vi "VIH - VI Doc Editor #2 - GenObject Symbols.vi"(6 "cmd (nop)":T2(ring), 8 "error in":errorcluster, 9 "type":enum16{"<Invalid>", "Control", "Page"}(ring), 11 "Gen Refnum":refnum<vi>) -> (0 "error out":errorcluster, 1 "Symbols":T1[](array[typedef]), 2 "Symbol Index":i32, 3 "dup Gen Refnum":refnum<vi>)   [LabVIEW 2014]
doc: "::: VI Helpeks :::\nCopyright (c) 2000-2026 Konstantin Shifershteyn. All rights reserved."
uses:
  <vilib>/picture/picture.llb/imagedata.ctl
panel:
  out "max Symbol Index":i32
  # "VI Helpeks\nCopyright (c) 2012-2026 Konstantin Shifershteyn"
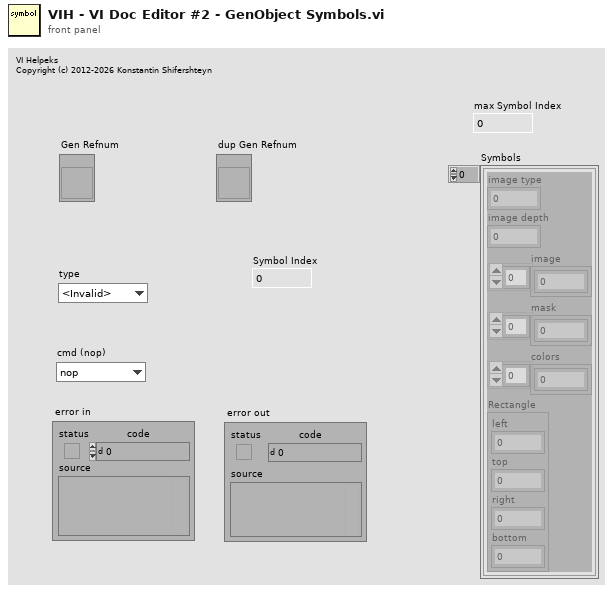
[diagram p1: front panel]
types:
  T1 = typedef "imagedata.ctl" = cluster{"image type":i32, "image depth":i32, "image":u8[], "mask":u8[], "colors":u32[], "Rectangle":cluster{"left":i16, "top":i16, "right":i16, "bottom":i16}}
  T2 = enum16{"nop", "Init", "get index", "get symbols"}
  T3 = cluster{"DefVal":variant, "Indicator":bool, i32}[]
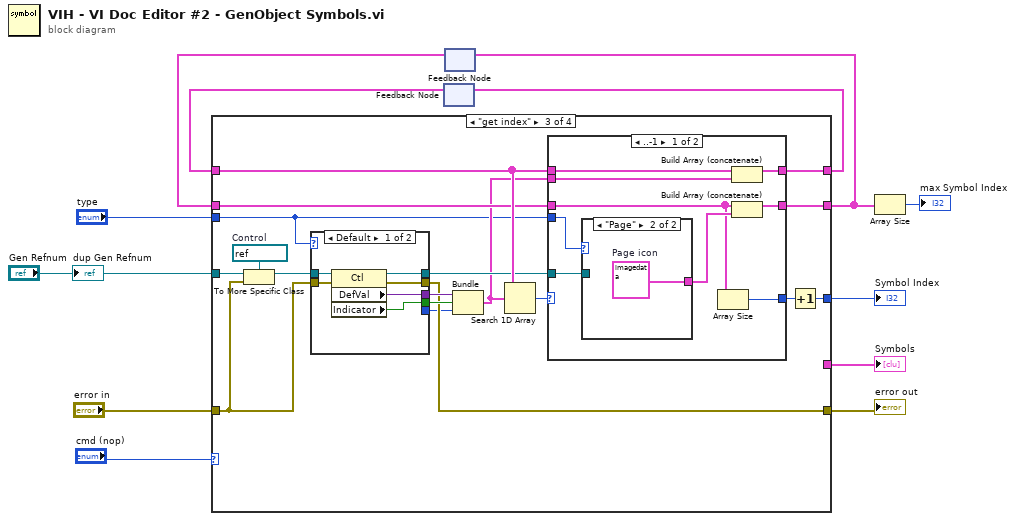
[diagram p0: block diagram]
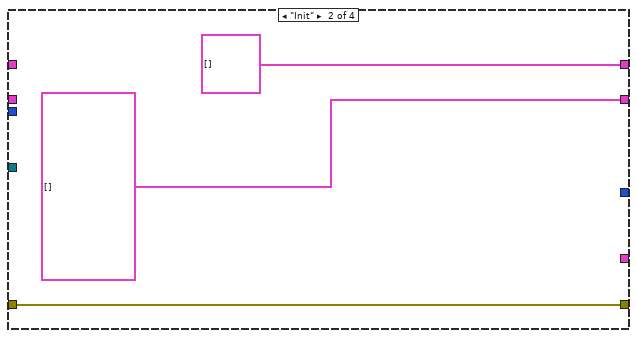
[diagram p3: hidden frame]
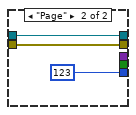
[diagram p4: hidden frame]
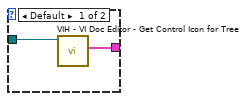
[diagram p5: hidden frame]
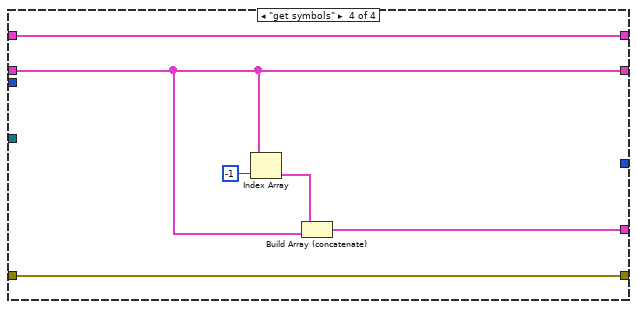
[diagram p7: hidden frame]
diagram:
  n1 = feedback #1() -> (w11:T3)  [unwired: 1 in]
  n2 = feedback #2() -> (w10:T1[])  [unwired: 1 in]
  n3 = case shown="\"get index\"" "cmd (nop)" {
    tunnel: [w15 T3 [] w36 w66] -> w12
    tunnel: w11 -> [w15 _ w35 w66]
    tunnel: w10 -> [w14 _ w34 w64]
    tunnel: [w14 T1[] [] w33 w64] -> w9
    tunnel: "Gen Refnum" -> [_ _ w22 _]
    tunnel: [_ _ w25 _] -> w7
    tunnel: [_ _ _ w62] -> w5
    tunnel: "error in" -> [w13 w17 w20 w61]
    tunnel: [w13 w17 w26 w61] -> w3
    tunnel: "type" -> [_ _ w19 _]
    frame "nop" {
    }
    frame "Init" {
    }
    frame "get index" {
      w23 = refnum<vi> refnum  # Control
      n4 = To More Specific Class(target class=w23, reference=w22, error in=w20) -> (specific class reference=w21:refnum<vi>)  [unwired: 1 out]
      n5 = case shown="Default" w19 {
        tunnel: [w42 w45] -> w31
        tunnel: [w41 _] -> w29
        tunnel: [w40 _] -> w28
        tunnel: [w39 w44] -> w26
        tunnel: w21 -> [w38 w45]
        tunnel: w20 -> [w37 w44]
        tunnel: [_ 123] -> w24
        frame Default {
          n6 = property class="Ctl"(reference=w38, error in=w37) -> (reference out=w42:refnum<vi>, error out=w39:errorcluster, "DefVal"=w41:variant, "Indicator"=w40:bool)
        }
        frame "Page" {
        }
      }
      n7 = Bundle("DefVal"=w29, "Indicator"=w28, w24) -> (w30:cluster{"DefVal":variant, "Indicator":bool, i32})  [unwired: 1 in]
      n8 = Search 1D Array(1D array=w35, element=w30) -> (index of element=w32:i32)  [unwired: 1 in]
      n9 = case shown="..-1" w32 {
        selector: w32 -> [_ w59]
        tunnel: [w53 w60] -> w36
        tunnel: w35 -> [w54 w60]
        tunnel: w30 -> [w52 _]
        tunnel: [w49 w59] -> w27
        tunnel: [w48 w58] -> w33
        tunnel: w34 -> [w47 w58]
        tunnel: w31 -> [w51 _]
        tunnel: w19 -> [w46 _]
        frame ..-1 {
          n10 = case shown="\"Page\"" w46 {
            tunnel: w51 -> [w56 _]
            tunnel: [w55 w57] -> w50
            frame Default {
              n11 = call "VIH - VI Doc Editor - Get Control Icon for Tree.vi"("Ctl Refnum"=w56) -> ("Icon"=w55:T1)  [unwired: 6 in, 4 out]
            }
            frame "Page" {
              w57 = T1 {"image type"=0, "image depth"=24, "image"=array[3072 elements], "mask"=[63, 254, 0, 0, 63, 255, 0, 0, 127, 255, 128, 0, 127, 255, 128, 0, 255, 255, 255, 252, 255, 255, 255, 254, 255, 255, 255, 255, 255, 255, 255, 255, 255, 255, 255, 255, 255, 255, 255, 255, 255, 255, 255, 255, 255, 255, 255, 255, 255, 255, 255, 255, 255, 255, 255, 255, 255, 255, 255, 255, 255, 255, 255, 255, 255, 255, 255, 255, 255, 255, 255, 255, 255, 255, 255, 255, 255, 255, 255, 255, 255, 255, 255, 255, 255, 255, 255, 255, 255, 255, 255, 255, 127, 255, 255, 254, 0, 0, 0, 0, 0, 0, 0, 0, 0, 0, 0, 0, 0, 0, 0, 0, 0, 0, 0, 0, 0, 0, 0, 0, 0, 0, 0, 0, 0, 0, 0, 0], "colors"=[], "Rectangle"={"left"=0, "top"=0, "right"=32, "bottom"=32}}  # Page icon
            }
          }
          n12 = Array Size(array=w47) -> (size(s)=w49:i32)
          n13 = Build Array (concatenate)(w54, w52) -> (w53:T3)
          n14 = Build Array (concatenate)(w47, w50) -> (w48:T1[])
        }
        frame 0.. {
        }
      }
      n15 = Increment(x=w27) -> (x+1=w25:i32)
    }
    frame "get symbols" {
      n16 = Index Array(array=w64, index=-1) -> (element=w63:T1)
      n17 = Build Array (concatenate)(w63, w64) -> (w62:T1[])
    }
  }
  "error out" <- w3
  "Symbol Index" <- w7
  "Symbols" <- w5
  n18 = feedback-in #1(w12) -> ()
  n19 = feedback-in #2(w9) -> ()
  n20 = Array Size(array=w9) -> (size(s)=→"max Symbol Index":i32)
  "dup Gen Refnum" <- "Gen Refnum"
